vi "addChild.vi"(0 "reference":refnum<class "AbstractNode.lvclass">, 1 "node":refnum<class "AbstractNode.lvclass">, 2 "index(last)":i32=-1, 5 "error in (no error)":errorcluster) -> (14 "reference out":refnum<class "AbstractNode.lvclass">, 19 "error out":errorcluster)   [LabVIEW 2020, in "AbstractNode.lvclass"]
doc: "public void addChild(int index, Node node)"
uses:
  <resource>/Framework/Providers/Open_GDS/UML/AbstractNode_class/AbstractNode.lvclass
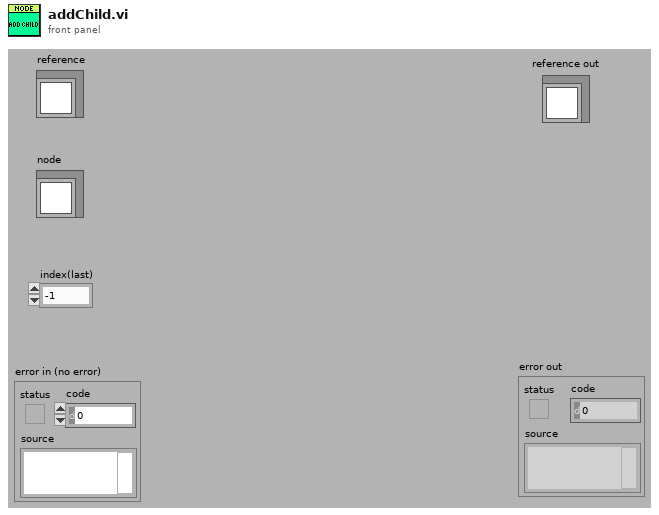
[diagram p1: front panel]
types:
  T1 = typedef "AbstractNode.lvclass/ObjectAttributes.ctl" = cluster{"parent":refnum<class "AbstractNode.lvclass">, "children":refnum<class "AbstractNode.lvclass">[], "Hidden":bool}
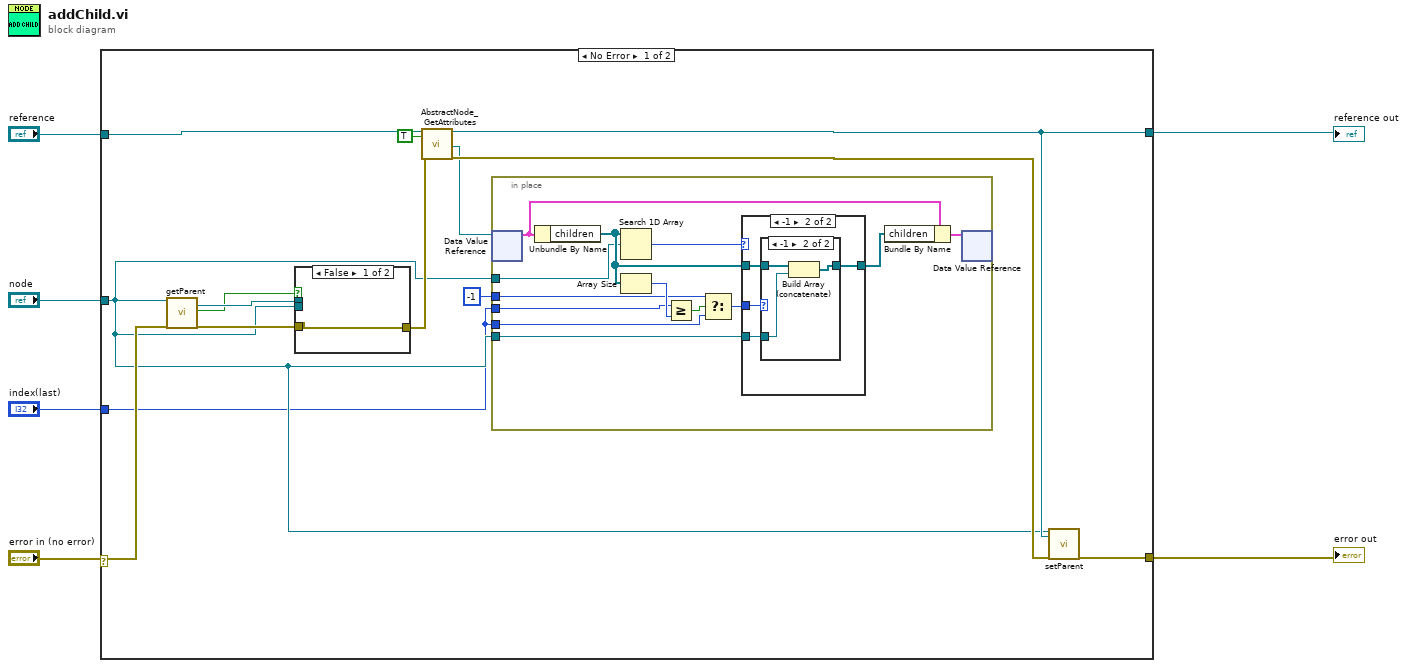
[diagram p0: block diagram]
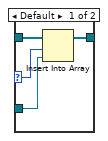
[diagram p3: hidden frame]
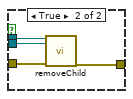
[diagram p4: hidden frame]
diagram:
  n1 = case shown="No Error" "error in (no error)" {
    selector: "error in (no error)" -> [w17 w51]
    tunnel: "reference" -> [w20 w52]
    tunnel: [w19 w51] -> w5
    tunnel: [w18 w52] -> w4
    tunnel: "node" -> [w9 _]
    tunnel: "index(last)" -> [w8 _]
    frame No Error {
      n2 = call-dynamic "getParent.vi"("reference"=w9, "error in (no error)"=w17) -> ("parentNode"=w13:refnum<class "AbstractNode.lvclass">, "ValidParent"=w12:bool, "error out"=w16:errorcluster)  [unwired: 13 in, 2 out]
      n3 = case shown="False" w12 {
        tunnel: w16 -> [w46 w50]
        tunnel: w13 -> [_ w49]
        tunnel: w9 -> [_ w48]
        tunnel: [w46 w47] -> w15
        frame False {
        }
        frame True {
          n4 = call-dynamic "removeChild.vi"("reference"=w49, "node"=w48, "error in (no error)"=w50) -> ("error out"=w47:errorcluster)  [unwired: 15 in, 1 out]
        }
      }
      n5 = call <resource>:"AbstractNode_GetAttributes.vi"("reference in"=w20, "OnlyGetDvrReference(False)"=TRUE, "error in (no error)"=w15) -> ("reference out"=w18:refnum<class "AbstractNode.lvclass">, "DataRef"=w10:refnum<data-value>, "error out"=w14:errorcluster)  [unwired: 13 in, 1 out]
      n6 = in-place {
        in-place-border: w9 -> [w28]
        in-place-border: w9 -> [w25]
        in-place-border: w8 -> [w24]
        in-place-border: w8 -> [w22]
        in-place-border: -1 ("t") -> [w21]
        n7 = in-place-dvr #1(w10) -> (w33:T1)  [unwired: 1 out]
        n8 = Unbundle By Name(w33) -> ("children"=w32:refnum<class "AbstractNode.lvclass">[])
        n9 = Search 1D Array(1D array=w32, element=w28) -> (index of element=w27:i32)  [unwired: 1 in]
        n10 = Array Size(array=w32) -> (size(s)=w29:i32)
        n11 = Greater Or Equal?(x=w24, y=w29) -> (x >= y?=w23:bool)
        n12 = Select(t=w21, s=w23, f=w22) -> (s? t:f=w26:i32)
        n13 = case shown="-1" w27 {
          tunnel: [w34 w38] -> w31
          tunnel: w26 -> [_ w37]
          tunnel: w32 -> [w34 w36]
          tunnel: w25 -> [_ w35]
          frame Default {
          }
          frame -1 {
            n14 = case shown="-1" w37 {
              selector: w37 -> [w40 _]
              tunnel: w36 -> [w42 w45]
              tunnel: [w41 w43] -> w38
              tunnel: w35 -> [w39 w44]
              frame Default {
                n15 = Insert Into Array(array=w42, index=w40, new element=w39) -> (w41:refnum<class "AbstractNode.lvclass">[])
              }
              frame -1 {
                n16 = Build Array (concatenate)(w45, w44) -> (w43:refnum<class "AbstractNode.lvclass">[])
              }
            }
          }
        }
        n17 = Bundle By Name(cluster=w33, "children"=w31) -> (w30:T1)
        n18 = in-place-dvr #1(w30) -> ()  [unwired: 2 out]
      }
      n19 = call-dynamic "setParent.vi"("reference"=w9, "node"=w18, "error in (no error)"=w14) -> ("error out"=w19:errorcluster)  [unwired: 15 in, 1 out]
    }
    frame Error {
    }
  }
  "reference out" <- w4
  "error out" <- w5
